vi "ActionVIOnCompile.vi"(8 "error in (no error)":errorcluster, 11 "Device Item Ref in":T4 format="%.0x") -> (0 "error out":errorcluster)   [LabVIEW 2020, in "SLSC EDS System Explorer.lvlib"]
uses:
  SLSC EDS System Explorer.lvlib
  <vilib>/NI VeriStand/Custom Device API/Custom Device Item Ref.ctl
  SLSC CD API/SLSC CD Engine/SLSC Dynamic Channel.ctl
  SLSC CD API/SLSC CD Engine/SLSC Datatype.ctl
  Shared/Compiled.Settings.ctl
  Shared/SLSC Static Settings.ctl
  Shared/Constants.vi
  <vilib>/NI VeriStand/Custom Device API/Get Item Property (Boolean).vi
  <vilib>/NI VeriStand/Custom Device Tools/Custom Device Utility Library/NI VeriStand - Search for Item by Name.vi
  <vilib>/NI VeriStand/Custom Device API/Get Item Property (I32).vi
  <vilib>/NI VeriStand/Custom Device API/Get Item Property (String).vi
  <vilib>/NI VeriStand/Custom Device Tools/Custom Device Utility Library/NI VeriStand - Search for All Items by Name.vi
  <vilib>/NI VeriStand/Custom Device API/Set Item Property (Variant).vi
  <vilib>/NI VeriStand/Custom Device Tools/Custom Device Utility Library/Custom Device Utility Library.lvlib
  <vilib>/NI VeriStand/Custom Device API/Custom Device API.lvlib
  <vilib>/NI/NIVS Inline Async API/_Data Access System Explorer/Data Access System Explorer.lvlib
  Shared/SLSC EDS Shared.lvlib
  SLSC CD API/SLSC CD Shared/SLSC CD Shared.lvlib
  SLSC CD API/SLSC CD System Explorer/SLSC CD System Explorer.lvlib
panel:
  out "appended array":T1(array[cluster])
  out "SLSC Commands":T2[](array[typedef])
  out "SLSC Set/Write Properties":T2[](array[typedef])
  out "SLSC Get/Read Properties":T2[](array[typedef])
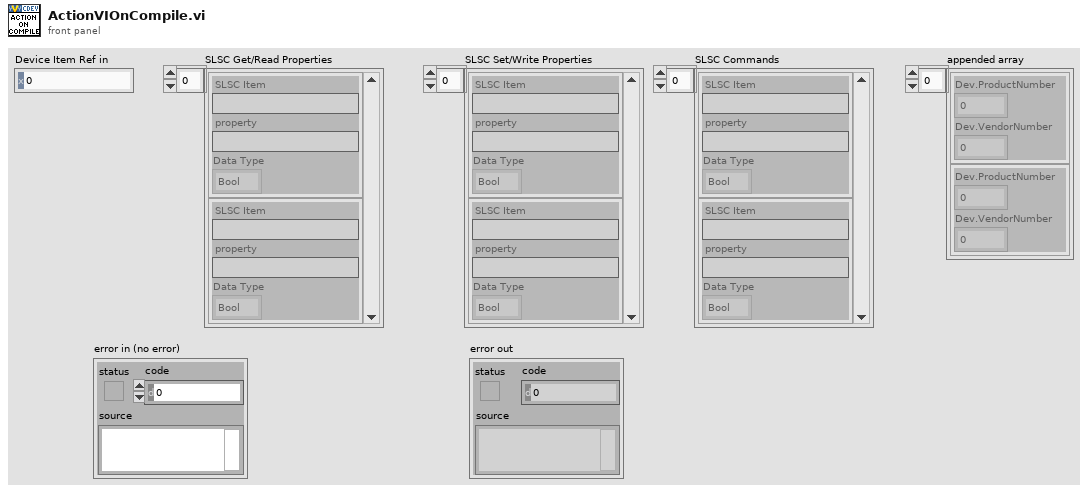
[diagram p1: front panel]
types:
  T1 = cluster{"Dev.ProductNumber":u32, "Dev.VendorNumber":u32}[]
  T2 = typedef "SLSC CD Shared.lvlib/SLSC Dynamic Channel.ctl" = cluster{"SLSC Item":string, "property":string, "Data Type":T3}
  T3 = typedef "SLSC CD Shared.lvlib/SLSC Datatype.ctl" = enum16{"Bool", "Double", "I32", "I64", "String", "U32", "U64"}
  T4 = typedef "Custom Device API.lvlib/Custom Device Item Ref.ctl" = u64
  T5 = cluster{"Dev.ProductNumber":u32, "Dev.VendorNumber":u32}
  T6 = enum16{"Output/Write", "Input/Read", "Input/ReadWrite"}
  T7 = typedef "SLSC EDS Shared.lvlib/Compiled.Settings.ctl" = cluster{"Name":string, "SLSC Name or IP Address":string, "Slot #":i32, "Reservation Access":i32, "Reservation Group":string, "Configuration Data":T8, "SLSC Get/Read Properties":T2[], "SLSC Set/Write Properties":T2[], "SLSC Dynamic Commands":T2[], "Support Modules":cluster{"Dev.ProductNumber":u32, "Dev.VendorNumber":u32}[]}
  T8 = typedef "SLSC EDS Shared.lvlib/SLSC Static Settings.ctl" = cluster{"Properties":cluster{"Boolean Properties":cluster{"property":refnum<k21>, "Value":bool, "SLSC Item":refnum<k21>, "reset value":bool}[], "Double Properties":cluster{"property":refnum<k21>, "Double Write":dbl, "SLSC Item":refnum<k21>, "Double Reset Value":dbl}[], "I32 Properties":cluster{"property":refnum<k21>, "Int32 Write":i32, "SLSC Item":refnum<k21>, "Int32 Reset Value":i32}[], "I64 Properties":cluster{"property":refnum<k21>, "Int64 Write":i64, "SLSC Item":refnum<k21>, "Int64 Reset Value":i64}[], "String Properties":cluster{"property":refnum<k21>, "String Write":string, "SLSC Item":refnum<k21>, "String Reset Value":string}[], "U32 Properties":cluster{"property":refnum<k21>, "UInt32 Write":u32, "SLSC Item":refnum<k21>, "UInt32 Reset Value":u32}[], "U64 Properties":cluster{"property":refnum<k21>, "UInt64 Write":u64, "SLSC Item":refnum<k21>, "UInt64 Reset Value":u64}[]}, "Commands":T2[], "Reset Commands":T2[], "Apply Values on Deployment":bool, "Apply Reset on Undeployment":bool, "Change Commands":T2[]}
  T9 = cluster{"Name":string, "Type":enum16{"Output/Write", "Input/Read", "Input/ReadWrite"}, "VS Refs":T4[]}
  T10 = typedef "Custom Device API.lvlib/Custom Device Item Info.ctl" = cluster{"Name":string, "Is Channel":bool, "GUID":string, "Is Waveform":bool}
  T11 = typedef "EDSjsonStructure.ctl" = cluster{"vendorNum":u32, "vendorName":string, "vendorPrefix":string, "productNum":u32, "productName":string, "capsVersion":string, "capsSpecVersion":u32, "capsSpecOldestCompatibleVersion":u32, "enums":T12[], "properties":T13[], "commands":T14[], "scales":T15[], "physicalChannels":T16[], "registerMap":cluster{"registers":T17[]}}
  T12 = typedef "enum.ctl" = cluster{"name":string, "description-en":string, "values":cluster{"name":string, "description-en":string, "value":i32}[]}
  T13 = typedef "property.ctl" = cluster{"name":string, "description-en":string, "documentation-en":string, "dataType":string, "bitfield":string, "access":string, "scale":string, "value":variant, "min":variant, "max":variant, "default value":variant}
  T14 = typedef "command.ctl" = cluster{"name":string, "description-en":string, "documentation-en":string, "startBitfield":string, "waitTimeInMs":i32, "doneBitfield":string, "doneInterrupt":string, "doneTimeoutInMs":i32, "value":variant}
  T15 = typedef "scale.ctl" = cluster{"name":string, "description-en":string, "m":dbl, "b":dbl, "forwardCoeffs":dbl[], "reverseCoeffs":dbl[], "coercion":string, "table":cluster{"scaled":dbl, "unscaled":dbl}[]}
  T16 = typedef "physicalChannel.ctl" = cluster{"name":string, "description-en":string, "commands":T14[], "properties":T13[]}
  T17 = typedef "register.ctl" = cluster{"name":string, "description-en":string, "access":string, "address":u32, "size":u32, "bitfields":cluster{"name":string, "description-en":string, "offset":u32, "size":u32, "signed":bool, "strobe":bool}[]}
  T18 = cluster{"Name":string, "Type":enum16{"Output/Write", "Input/Read", "Input/ReadWrite"}, "VS Refs":T4[]}[]
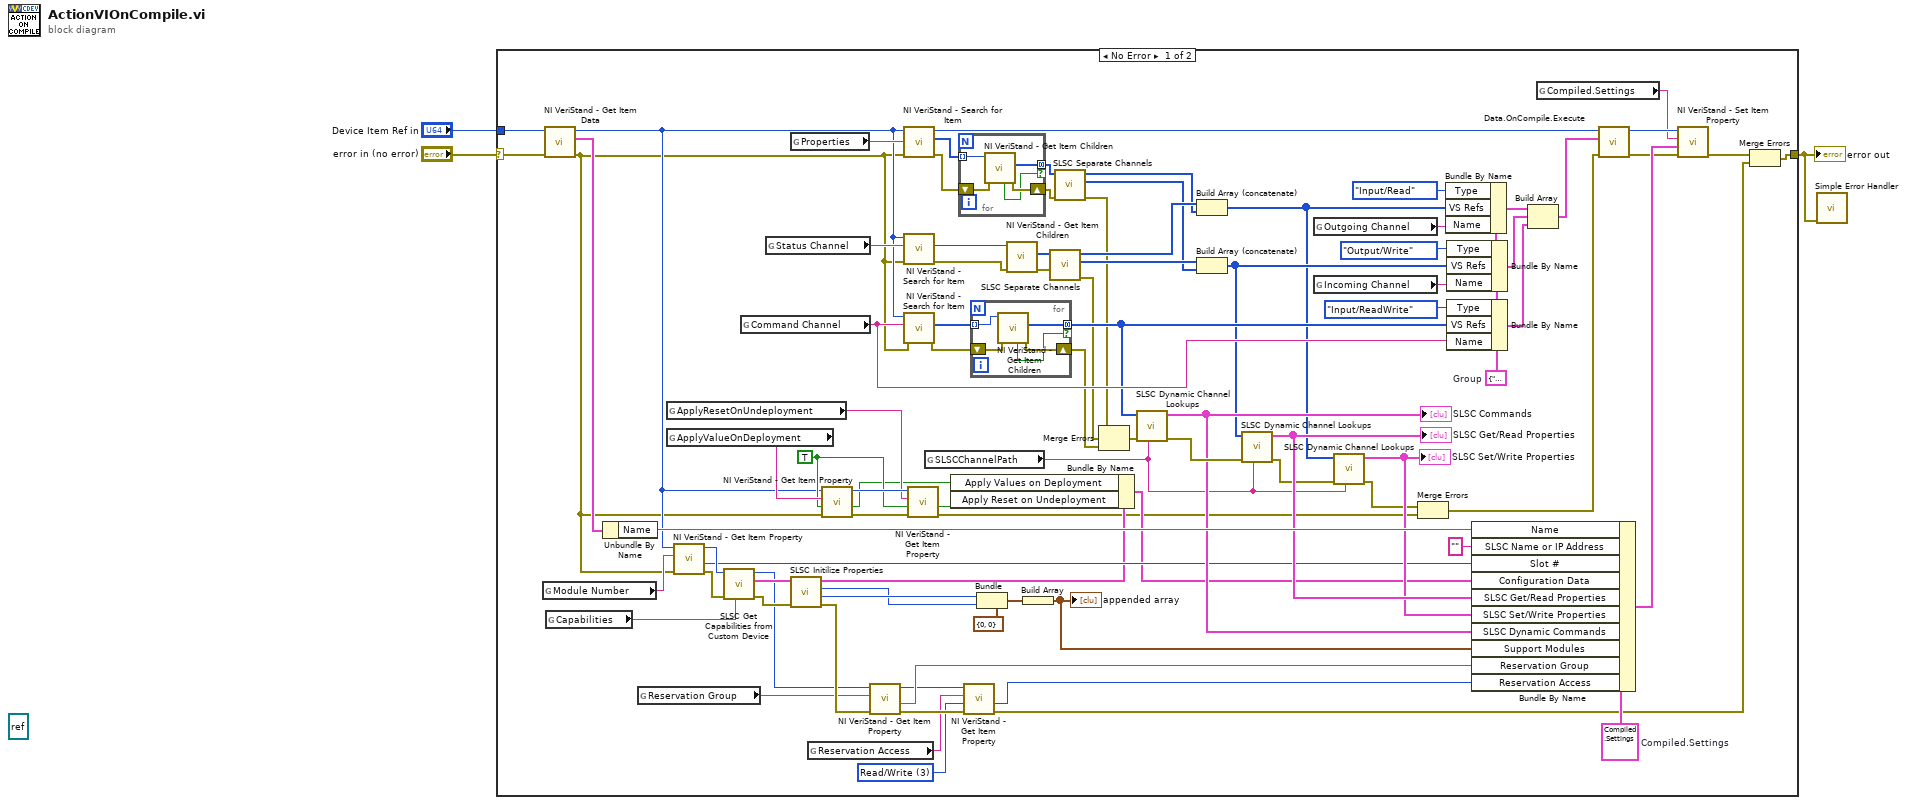
[diagram p0: block diagram]
diagram:
  (unwired) refnum<k7> refnum ("SHDocVw.IWebBrowser2")
  n1 = case shown="No Error" "error in (no error)" {
    selector: "error in (no error)" -> [w78 w103]
    tunnel: [w76 w103] -> w1
    tunnel: "Device Item Ref in" -> [w79 _]
    frame No Error {
      w4 = 3 items=["None"=0, "Read Only"=1, "Read/Write"=3] ("reservation access (Read/Write)")
      w25 = TRUE ("Default Value")
      w71 = T7 {"Name"="", "SLSC Name or IP Address"="", "Slot #"=0, "Reservation Access"=3, "Reservation Group"="", "Configuration Data"={"Properties"={"Boolean Properties"=[], "Double Properties"=[], "I32 Properties"=[], "I64 Properties"=[], "String Properties"=[], "U32 Properties"=[], "U64 Properties"=[]}, "Commands"=[], "Reset Commands"=[], "Apply Values on Deployment"=TRUE, "Apply Reset on Undeployment"=TRUE, "Change Commands"=[]}, "SLSC Get/Read Properties"=[], "SLSC Set/Write Properties"=[], "SLSC Dynamic Commands"=[], "Support Modules"=[]}  # Compiled.Settings
      w63 = T9 {"Name"="", "Type"=enum."Output/Write", "VS Refs"=[]}  # Group
      n2 = global read "Constants.vi" "Module Number"() -> (w80:string)
      n3 = call <vilib>:"NI VeriStand - Get Item Data.vi"("error in (no error)"=w78, "Item Ref in"=w79) -> ("error out"=w19:errorcluster, "Item Info"=w89:T10, "Item Ref out"=w24:T4)  [unwired: 6 in, 1 out]
      n4 = global read "Constants.vi" "Capabilities"() -> (w15:string)
      n5 = Unbundle By Name(w89) -> ("Name"=w88:string)
      n6 = global read "Constants.vi" "Reservation Group"() -> (w12:string)
      n7 = global read "Constants.vi" "ApplyResetOnUndeployment"() -> (w27:string)
      n8 = global read "Constants.vi" "ApplyValueOnDeployment"() -> (w29:string)
      n9 = call-poly <vilib>:"NI VeriStand - Get Item Property.vi"("error in (no error)"=w19, "Property Name"=w80, "Item Ref in"=w24) -> ("error out"=w32:errorcluster, "Value"=w33:i32, "Item Ref out"=w35:T4)  [unwired: 5 in, 1 out]
      n10 = call "SLSC Get Capabilities from Custom Device.vi"("Property Name"=w15, "error in (no error)"=w32, "Device Item Ref in"=w35) -> ("error out"=w31:errorcluster, "data"=w34:T11, "Item Ref out"=w11:T4)  [unwired: 3 in, 3 out]
      n11 = global read "Constants.vi" "Command Channel"() -> (w64:string)
      n12 = global read "Constants.vi" "Status Channel"() -> (w68:string)
      n13 = global read "Constants.vi" "Properties"() -> (w73:string)
      n14 = call "SLSC Initilize Properties.vi"("error in (no error)"=w31, "Capabilities"=w34) -> ("error out"=w13:errorcluster, "productNum"=w36:u32, "vendorNum"=w30:u32, "Configuration Data"=w23:T8)  [unwired: 5 in, 1 out]
      n15 = global read "Constants.vi" "Reservation Access"() -> (w7:string)
      n16 = call-poly <vilib>:"NI VeriStand - Get Item Property.vi"("error in (no error)"=w19, "Default Value"=w25, "Property Name"=w29, "Item Ref in"=w24) -> ("error out"=w26:errorcluster, "Value"=w21:bool, "Item Ref out"=w28:T4)  [unwired: 4 in, 1 out]
      n17 = call-poly <vilib>:"NI VeriStand - Get Item Property.vi"("error in (no error)"=w13, "Property Name"=w12, "Item Ref in"=w11) -> ("error out"=w8:errorcluster, "Value"=w10:string, "Item Ref out"=w6:T4)  [unwired: 5 in, 1 out]
      n18 = call-poly <vilib>:"NI VeriStand - Search for Item.vi"("error in"=w19, "Item Name"=w73, "Section Ref in"=w24) -> ("error out"=w45:errorcluster, "Item Refs"=w92:T4[], "Section Ref out"=w53:T4)  [unwired: 5 in, 1 out]
      n19 = call-poly <vilib>:"NI VeriStand - Search for Item.vi"("error in"=w19, "Item Name"=w68, "Section Ref in"=w24) -> ("error out"=w70:errorcluster, "Item Ref"=w69:T4)  [unwired: 5 in, 2 out]
      n20 = call-poly <vilib>:"NI VeriStand - Search for Item.vi"("error in"=w19, "Item Name"=w64, "Section Ref in"=w24) -> ("error out"=w66:errorcluster, "Item Refs"=w67:T4[])  [unwired: 5 in, 2 out]
      n21 = call-poly <vilib>:"NI VeriStand - Get Item Property.vi"("error in (no error)"=w26, "Default Value"=w25, "Property Name"=w27, "Item Ref in"=w28) -> ("error out"=w17:errorcluster, "Value"=w20:bool)  [unwired: 4 in, 2 out]
      n22 = global read "Constants.vi" "SLSCChannelPath"() -> (w16:string)
      n23 = Bundle By Name(cluster=w23, "Apply Values on Deployment"=w21, "Apply Reset on Undeployment"=w20) -> (w22:T8)
      n24 = for {
        tunnel: w92 -> [w97] mode=indexing
        tunnel: [w95] -> w52 mode=concatenating if=w93
        shift-right: [w94] -> w47
        shift-left: w45 -> [w96]
        n25 = call <vilib>:"NI VeriStand - Get Item Children.vi"("error in (no error)"=w96, "Item Ref in"=w97) -> ("error out"=w94:errorcluster, "Child Refs"=w95:T4[], "Found"=w93:bool)  [unwired: 6 in, 1 out]
      }
      n26 = call-poly <vilib>:"NI VeriStand - Get Item Property.vi"("error in (no error)"=w8, "Default Value"=w4, "Property Name"=w7, "Item Ref in"=w6) -> ("error out"=w9:errorcluster, "Value"=w5:i32)  [unwired: 4 in, 2 out]
      n27 = for {
        tunnel: w67 -> [w102] mode=indexing
        tunnel: [w99] -> w58 mode=concatenating if=w98
        shift-right: [w100] -> w62
        shift-left: w66 -> [w101]
        n28 = call <vilib>:"NI VeriStand - Get Item Children.vi"("error in (no error)"=w101, "Item Ref in"=w102) -> ("error out"=w100:errorcluster, "Child Refs"=w99:T4[], "Found"=w98:bool)  [unwired: 6 in, 1 out]
      }
      n29 = Bundle(cluster=T5 {"Dev.ProductNumber"=0, "Dev.VendorNumber"=0} ("Product Identification"), "Dev.ProductNumber"=w36, "Dev.VendorNumber"=w30) -> (w38:T5)
      n30 = call <vilib>:"NI VeriStand - Get Item Children.vi"("error in (no error)"=w70, "Item Ref in"=w69) -> ("error out"=w46:errorcluster, "Child Refs"=w56:T4[])  [unwired: 6 in, 2 out]
      n31 = Build Array(w38) -> (w37:T1)
      "appended array" <- w37
      n32 = call "SLSC Separate Channels.vi"("error in (no error)"=w46, "Item Refs In"=w56) -> ("error out"=w43:errorcluster, "Output Channels"=w54:T4[], "Input Channels"=w55:T4[])  [unwired: 6 in, 1 out]
      n33 = call "SLSC Separate Channels.vi"("error in (no error)"=w47, "Item Refs In"=w52) -> ("error out"=w42:errorcluster, "Output Channels"=w50:T4[], "Input Channels"=w51:T4[])  [unwired: 6 in, 1 out]
      n34 = Merge Errors(w42, w43, w62) -> (w60:errorcluster)
      n35 = call "SLSC Dynamic Channel Lookups.vi"("SLSCChannelPath"=w16, "error in (no error)"=w60, "Child Refs"=w58) -> ("error out"=w59:errorcluster, "SLSC Dynamic Inputs"=w57:T2[])  [unwired: 7 in]
      "SLSC Commands" <- w57
      n36 = Build Array (concatenate)(w55, w51) -> (w40:T4[])
      n37 = Build Array (concatenate)(w54, w50) -> (w41:T4[])
      n38 = call "SLSC Dynamic Channel Lookups.vi"("SLSCChannelPath"=w16, "error in (no error)"=w59, "Child Refs"=w41) -> ("error out"=w74:errorcluster, "SLSC Dynamic Inputs"=w75:T2[])  [unwired: 7 in]
      "SLSC Get/Read Properties" <- w75
      n39 = global read "Constants.vi" "Outgoing Channel"() -> (w49:string)
      n40 = global read "Constants.vi" "Incoming Channel"() -> (w48:string)
      n41 = call "SLSC Dynamic Channel Lookups.vi"("SLSCChannelPath"=w16, "error in (no error)"=w74, "Child Refs"=w40) -> ("error out"=w44:errorcluster, "SLSC Dynamic Inputs"=w72:T2[])  [unwired: 7 in]
      "SLSC Set/Write Properties" <- w72
      n42 = Merge Errors(w44, w17) -> (w18:errorcluster)
      n43 = Bundle By Name(cluster=w63, "Type"=T6."Input/Read", "VS Refs"=w40, "Name"=w49) -> (w87:T9)
      n44 = Bundle By Name(cluster=w63, "Type"=T6."Output/Write", "VS Refs"=w41, "Name"=w48) -> (w83:T9)
      n45 = Bundle By Name(cluster=w63, "Type"=T6."Input/ReadWrite", "VS Refs"=w58, "Name"=w64) -> (w61:T9)
      n46 = Bundle By Name(cluster=w71, "Name"=w88, "SLSC Name or IP Address"="", "Slot #"=w33, "Configuration Data"=w22, "SLSC Get/Read Properties"=w75, "SLSC Set/Write Properties"=w72, "SLSC Dynamic Commands"=w57, "Support Modules"=w37, "Reservation Group"=w10, "Reservation Access"=w5) -> (w91:T7)
      n47 = Build Array(w87, w83, w61) -> (w85:T18)
      n48 = global read "Constants.vi" "Compiled.Settings"() -> (w77:string)
      n49 = call <vilib>:"Data.OnCompile.Execute.vi"("error in"=w18, "VS Ref Groups"=w85, "Custom Device Ref"=w53) -> ("error out"=w82:errorcluster, "Custom Device Ref"=w81:T4)  [unwired: 7 in]
      n50 = call-poly <vilib>:"NI VeriStand - Set Item Property.vi"("error in (no error)"=w82, "Value"=w91, "Property Name"=w77, "Item Ref in"=w81) -> ("error out"=w90:errorcluster)  [unwired: 5 in, 2 out]
      n51 = Merge Errors(w90, w9) -> (w76:errorcluster)
    }
    frame Error {
    }
  }
  "error out" <- w1
  n52 = call <vilib>:"Simple Error Handler.vi"("error in (no error)"=w1) -> ()  [unwired: 4 in, 5 out]
